vi "VIH Project - Container - Project File Path.vi"(7 "cmd (get)":enum16{"get", "set"}(ring), 11 "Project File Path in":path) -> (2 "Project Build Log File":path, 3 "Project File Path":path, 5 "It's example":bool)   [LabVIEW 2014]
doc: "::: VI Helpeks :::\nCopyright (c) 2000-2026 Konstantin Shifershteyn. All rights reserved."
panel:
  # "VI Helpeks\nCopyright (c) 2012-2026 Konstantin Shifershteyn"
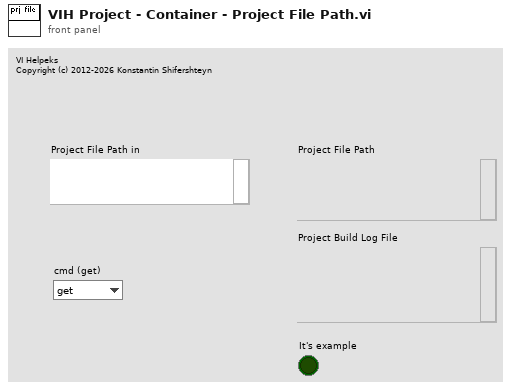
[diagram p1: front panel]
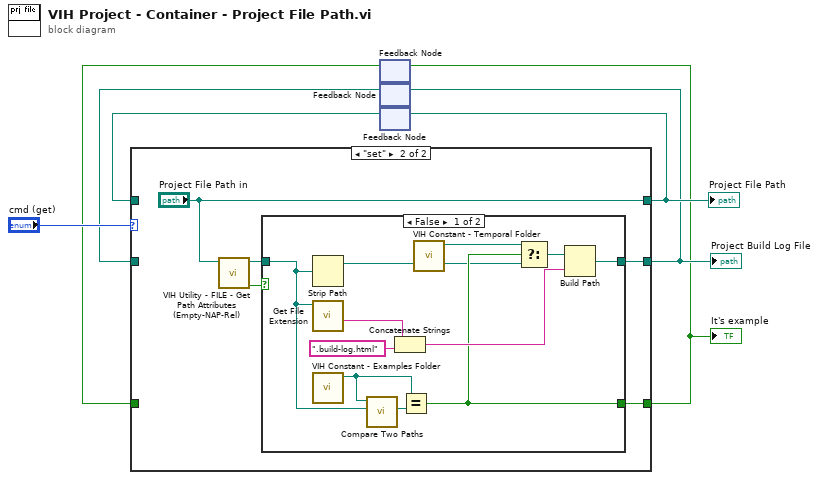
[diagram p0: block diagram]
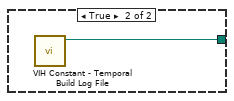
[diagram p3: hidden frame]
diagram:
  n1 = feedback #1() -> (w2:bool)  [unwired: 1 in]
  n2 = feedback #2() -> (w4:path)  [unwired: 1 in]
  n3 = feedback #3() -> (w5:path)  [unwired: 1 in]
  n4 = case shown="\"set\"" "cmd (get)" {
    tunnel: [w10 "Project File Path in"] -> w6
    tunnel: w5 -> [w10 _]
    tunnel: [w9 w15] -> w3
    tunnel: w4 -> [w9 _]
    tunnel: [w8 w11] -> w1
    tunnel: w2 -> [w8 _]
    frame "get" {
    }
    frame "set" {
      n5 = call "VIH Utility - FILE - Get Path Attributes (Empty-NAP-Rel).vi"("Path"="Project File Path in") -> ("Not A Path or Empty path"=w12:bool, "dup Path"=w14:path)  [unwired: 6 in, 3 out]
      n6 = case shown="False" w12 {
        tunnel: [w23 w27] -> w15
        tunnel: w14 -> [w22 _]
        tunnel: [w18 _] -> w11
        frame False {
          n7 = Strip Path(path=w22) -> (stripped path=w17:path)  [unwired: 1 out]
          n8 = call <vilib>:"Get File Extension.vi"("file"=w22) -> ("filename without extension"=w26:string)  [unwired: 7 in, 3 out]
          n9 = call "VIH Constant - Examples Folder.vi"() -> ("Examples folder"=w19:path)  [unwired: 11 in]
          n10 = call <vilib>:"Compare Two Paths.vi"("Path 2"=w22, "Path 1"=w19) -> ("Common Path"=w21:path)  [unwired: 6 in, 3 out]
          n11 = Concatenate Strings(w26, ".build-log.html" ("string")) -> (w24:string)
          n12 = Equal?(x=w19, y=w21) -> (x = y?=w18:bool)
          n13 = call "VIH Constant - Temporal Folder.vi"() -> ("Temporal folder"=w16:path)  [unwired: 11 in]
          n14 = Select(t=w16, s=w18, f=w17) -> (s? t:f=w20:path)
          n15 = Build Path(base path=w20, name or relative path=w24) -> (appended path=w23:path)
        }
        frame True {
          n16 = call "VIH Constant - Temporal Build Log File.vi"() -> ("Temporal Build Log File"=w27:path)  [unwired: 11 in]
        }
      }
    }
  }
  "Project File Path" <- w6
  "Project Build Log File" <- w3
  "It's example" <- w1
  n17 = feedback-in #1(w1) -> ()
  n18 = feedback-in #2(w3) -> ()
  n19 = feedback-in #3(w6) -> ()
